vi "Apply Task Rows.vi"(8 "error in":errorcluster, 9 "Task Rows":T1[](array[typedef]), 10 "Project ID":string, 11 "Project Store in":refnum<class "Project Store.lvclass">) -> (0 "error out":errorcluster, 3 "Project Store out":refnum<class "Project Store.lvclass">)   [LabVIEW 2026]
doc: "Applies edited Task Edit Row clusters {Task Name, Active} to one project and writes the Project Store to its data source once. Each Task Name is trimmed; empty names are skipped, and a name that appears twice is used only the first time. A name the project already has (exact match, active or inactive) gets the row's Active with Update Task when it differs. A new name is added with Add Task (new GUID, next Sort Order) and then given the row's Active. Tasks not in the rows are left alone and nothing is removed. An empty or unknown Project ID returns error 5102 (Apply Task Rows: project ID not found.) and writes nothing.\n\nInputs: Project Store in; Project ID; Task Rows; error in.\nOutputs: Project Store out; error out.\n\nGenerated by: Claude"
uses:
  Storage/Project Store/Project Store.lvclass
  Task Edit Row.ctl
  <vilib>/Utility/error.llb/Trim Whitespace One-Sided.vi
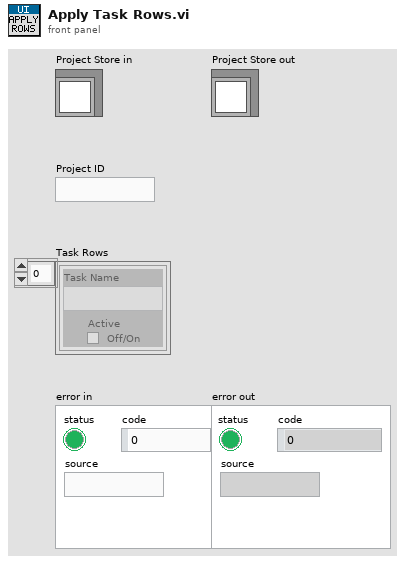
[diagram p1: front panel]
types:
  T1 = typedef "Task Edit Row.ctl" = cluster{"Task Name":string, "Active":bool}
  T2 = typedef "Task List.ctl" = T3[]
  T3 = typedef "Task.ctl" = cluster{"ID":string, "Project ID":string, "Name":string, "Active":bool, "Sort Order":i32}
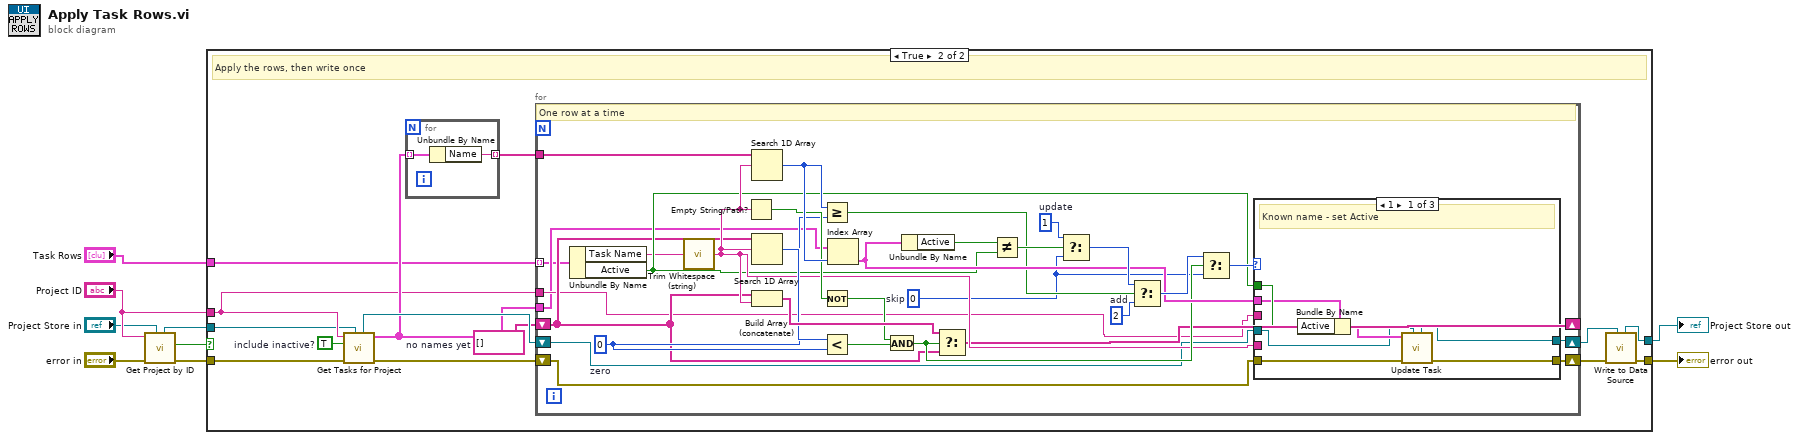
[diagram p0: block diagram]
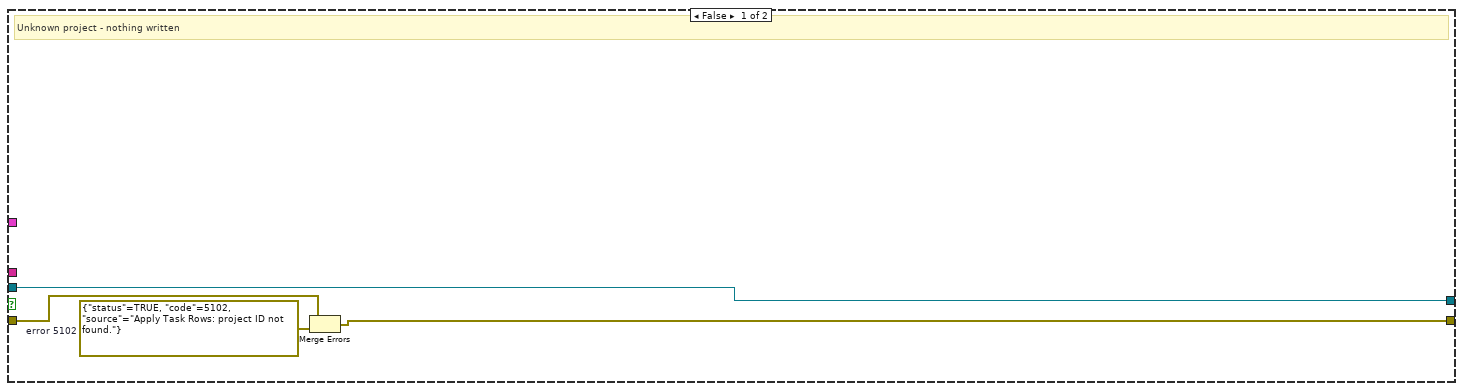
[diagram p2: hidden frame]
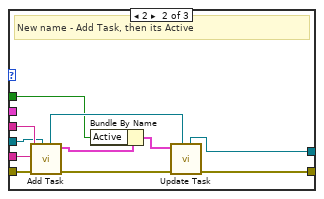
[diagram p3: hidden frame]
diagram:
  n1 = call-dynamic "Get Project by ID.vi"("Project Store in"="Project Store in", "error in (no error)"="error in", "ID"="Project ID") -> ("error out"=w7:errorcluster, "found?"=w8:bool, "Project Store out"=w9:refnum<class "Project Store.lvclass">)  [unwired: 5 in, 1 out]
  n2 = case shown="True" w8 {
    tunnel: "Project ID" -> [_ w16]
    tunnel: "Task Rows" -> [_ w17]
    tunnel: w9 -> [w10 w14]
    tunnel: w7 -> [w11 w15]
    tunnel: [w10 w18] -> w5
    tunnel: [w12 w19] -> w6
    frame False {
      w13 = errorcluster {"status"=TRUE, "code"=5102, "source"="Apply Task Rows: project ID not found."}  # error 5102
      # "Unknown project - nothing written"
      n3 = Merge Errors(w11, w13) -> (w12:errorcluster)
    }
    frame True {
      w21 = string[] []  # no names yet
      w20 = TRUE  # include inactive?
      # "Apply the rows, then write once"
      n4 = call-dynamic "Get Tasks for Project.vi"("Project Store in"=w14, "error in (no error)"=w15, "include inactive?"=w20, "Project ID"=w16) -> ("error out"=w22:errorcluster, "Tasks"=w23:T2, "Project Store out"=w24:refnum<class "Project Store.lvclass">)  [unwired: 5 in]
      n5 = for {
        tunnel: w23 -> [w79] mode=indexing
        tunnel: [w80] -> w25 mode=indexing
        n6 = Unbundle By Name(w79) -> ("Name"=w80:string)
      }
      n7 = for {
        shift-right: [w37] -> _
        shift-left: w21 -> [w36]
        tunnel: w17 -> [w28] mode=indexing
        tunnel: w16 -> [w31]
        tunnel: w23 -> [w29]
        shift-right: [w33] -> w26
        shift-left: w24 -> [w32]
        shift-right: [w35] -> w27
        shift-left: w22 -> [w34]
        tunnel: w25 -> [w30]
        w41 = 2  # add
        w40 = 1  # update
        w39 = 0  # skip
        w38 = 0  # zero
        # "One row at a time"
        n8 = Unbundle By Name(w28) -> ("Task Name"=w42:string, "Active"=w43:bool)
        n9 = call <vilib>:"Trim Whitespace (string).vi"("string"=w42) -> ("trimmed string"=w44:string)  [unwired: 1 in]
        n10 = Empty String/Path?(string/path=w44) -> (empty?=w45:bool)
        n11 = Search 1D Array(1D array=w30, element=w44) -> (index of element=w50:i32)  [unwired: 1 in]
        n12 = Search 1D Array(1D array=w36, element=w44) -> (index of element=w47:i32)  [unwired: 1 in]
        n13 = Build Array (concatenate)(w36, w44) -> (w58:string[])
        n14 = Greater Or Equal?(x=w50, y=w38) -> (x >= y?=w51:bool)
        n15 = Not(x=w45) -> (.not. x?=w46:bool)
        n16 = Less?(x=w47, y=w38) -> (x < y?=w48:bool)
        n17 = Index Array(array=w29, index=w50) -> (element=w52:T3)
        n18 = And(x=w46, y=w48) -> (x .and. y?=w49:bool)
        n19 = Unbundle By Name(w52) -> ("Active"=w53:bool)
        n20 = Select(t=w58, s=w49, f=w36) -> (s? t:f=w37:string[])
        n21 = Not Equal?(x=w53, y=w43) -> (x != y?=w54:bool)
        n22 = Select(t=w40, s=w54, f=w39) -> (s? t:f=w55:i32)
        n23 = Select(t=w55, s=w51, f=w41) -> (s? t:f=w56:i32)
        n24 = Select(t=w56, s=w49, f=w39) -> (s? t:f=w57:i32)
        n25 = case shown="1" w57 {
          tunnel: w31 -> [_ w70 _]
          tunnel: w43 -> [w62 w68 _]
          tunnel: w32 -> [w59 w66 w77]
          tunnel: w34 -> [w60 w67 w78]
          tunnel: w44 -> [_ w69 _]
          tunnel: w52 -> [w61 _ _]
          tunnel: [w63 w71 w77] -> w33
          tunnel: [w64 w72 w78] -> w35
          frame 1 {
            # "Known name - set Active"
            n26 = Bundle By Name(cluster=w61, "Active"=w62) -> (w65:T3)
            n27 = call-dynamic "Update Task.vi"("Project Store in"=w59, "error in (no error)"=w60, "Task"=w65) -> ("error out"=w64:errorcluster, "Project Store out"=w63:refnum<class "Project Store.lvclass">)  [unwired: 6 in, 1 out]
          }
          frame 2 {
            # "New name - Add Task, then its Active"
            n28 = call-dynamic "Add Task.vi"("Project Store in"=w66, "error in (no error)"=w67, "Name"=w69, "Project ID"=w70) -> ("error out"=w73:errorcluster, "Task"=w74:T3, "Project Store out"=w75:refnum<class "Project Store.lvclass">)  [unwired: 5 in]
            n29 = Bundle By Name(cluster=w74, "Active"=w68) -> (w76:T3)
            n30 = call-dynamic "Update Task.vi"("Project Store in"=w75, "error in (no error)"=w73, "Task"=w76) -> ("error out"=w72:errorcluster, "Project Store out"=w71:refnum<class "Project Store.lvclass">)  [unwired: 6 in, 1 out]
          }
          frame Default {
            # "Empty, repeated or unchanged"
          }
        }
      }
      n31 = call-dynamic "Write to Data Source.vi"("Project Store in"=w26, "error in (no error)"=w27) -> ("error out"=w19:errorcluster, "Project Store out"=w18:refnum<class "Project Store.lvclass">)  [unwired: 8 in]
    }
  }
  "Project Store out" <- w5
  "error out" <- w6
